vi "BinLiftingSequence.vi"(0 "isAlreadyPickedUp":bool, 2 "NXT/EV3 IN":T1, 3 "Motor IDs":cluster{"Motors":T2, "Motors 2":T2}={"Motors"=0, "Motors 2"=1} {"Motors" items=["Port A", "Port B", "Port C", "Port D"]; "Motors 2" items=["Port A", "Port B", "Port C", "Port D"]}) -> (1 "IsHeavy":bool, 4 "alreadyPickedUp":bool, 5 "NXT/EV3 OUT":T1)   [LabVIEW 2016, in "13.03 Robot.lvrbt"]
uses:
  13.03 Robot.lvrbt
  <vilib>/NXT/Block Support/NXT_OutputPort.ctl
  <vilib>/NXT/Subs/LVHSConnector.ctl
  <vilib>/NXT/LegoClasses/BrickReference/BrickReference.lvclass
  <vilib>/NXT/NXTIO Xnodes/NXTIONodeSubVIs/NXTStopMotors.vi
  <vilib>/NXT/NXTIO Xnodes/NXTIOXNode/NXTIO.xnode
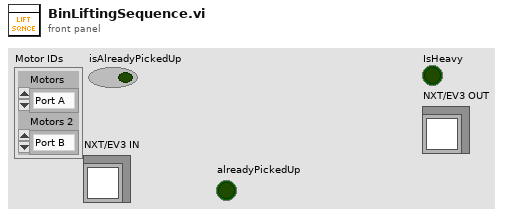
[diagram p1: front panel]
types:
  T1 = typedef "LVHSConnector.ctl" = refnum<class "BrickReference.lvclass">
  T2 = typedef "NXT_OutputPort.ctl" = u8
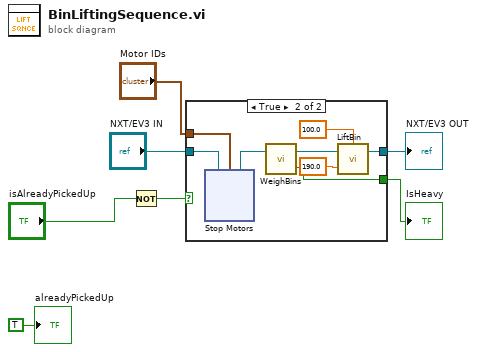
[diagram p0: block diagram]
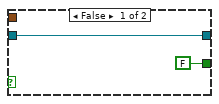
[diagram p2: hidden frame]
diagram:
  n1 = Not(x="isAlreadyPickedUp") -> (.not. x?=w3:bool)
  n2 = case shown="True" w3 {
    tunnel: "NXT/EV3 IN" -> [w8 w15]
    tunnel: [FALSE ("IsHeavy") w16] -> w7
    tunnel: "Motor IDs" -> [_ w12]
    tunnel: [w8 w11] -> w5
    frame False {
    }
    frame True {
      n3 = xnode "Stop Motors"("Motors"=w12, "NXT/EV3"=w15) -> ("NXT/EV3"=w14:T1)
      n4 = call "WeighBins.vi"("NXT/EV3 IN"=w14) -> ("IsHeavy"=w16:bool, "NXT/EV3 OUT"=w13:T1)  [unwired: 4 in]
      n5 = call "LiftBin.vi"("Position to Reach"=190.0, "NXT/EV3 IN"=w13, "Speed"=100.0) -> ("NXT/EV3 OUT"=w11:T1)
    }
  }
  "IsHeavy" <- w7
  "NXT/EV3 OUT" <- w5
  "alreadyPickedUp" <- TRUE ("alreadyPickedUp")
